vi "BSD Filename Header Formation.vi"(11 "Pre File F_Name":string) -> (3 "Head for BNAL":string)   [LabVIEW 2018]
panel:
  out "String":string
  out "Array":string[](array[string])
  out "after substring":string
  out "部分文字列の後":string
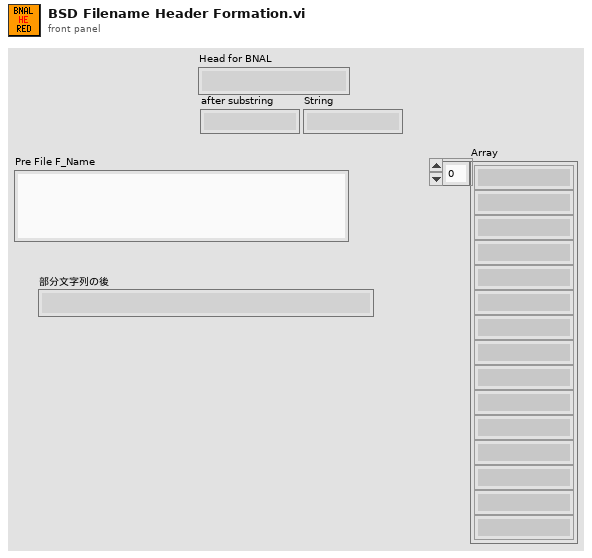
[diagram p1: front panel]
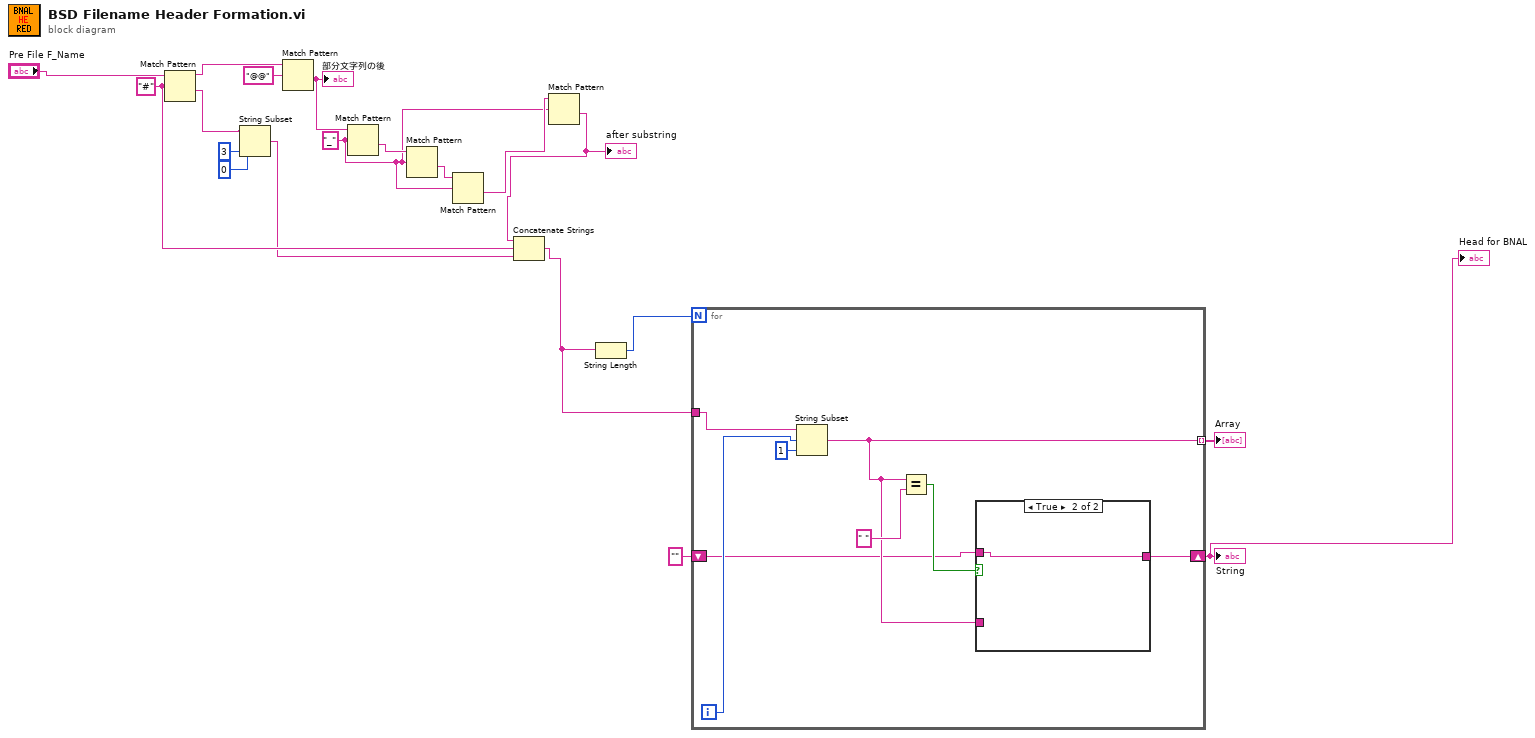
[diagram p0: block diagram]
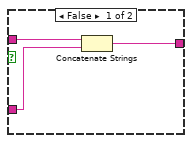
[diagram p2: hidden frame]
diagram:
  w7 = "_" ("正規表現")
  w10 = "#" ("正規表現")
  n1 = Match Pattern(string="Pre File F_Name", regular expression=w10) -> (before substring=w18:string, after substring=w13:string)  [unwired: 1 in, 2 out]
  n2 = String Subset(string=w13, offset (0)=0 ("オフセット（0）"), length (rest)=3 ("長さ（残り）")) -> (substring=w9:string)
  n3 = Match Pattern(string=w18, regular expression="@@" ("正規表現")) -> (after substring=w16:string)  [unwired: 1 in, 3 out]
  "部分文字列の後" <- w16
  n4 = Match Pattern(string=w16, regular expression=w7) -> (after substring=w15:string)  [unwired: 1 in, 3 out]
  n5 = Match Pattern(string=w15, regular expression=w7) -> (after substring=w14:string)  [unwired: 1 in, 3 out]
  n6 = Match Pattern(string=w14, regular expression=w7) -> (after substring=w8:string)  [unwired: 1 in, 3 out]
  n7 = Match Pattern(string=w8, regular expression=w7) -> (after substring=w6:string)  [unwired: 1 in, 3 out]
  "after substring" <- w6
  n8 = Concatenate Strings(w6, w10, w9) -> (w4:string)
  n9 = String Length(string=w4) -> (length=w5:i32)
  n10 = for {
    N: w5 -> [_]
    tunnel: w4 -> [w25]
    tunnel: [w22] -> w3 mode=indexing
    shift-right: [w21] -> w1
    shift-left: "" -> [w20]
    i -> [w26]
    n11 = String Subset(string=w25, offset (0)=w26, length (rest)=1 ("length (rest)")) -> (substring=w22:string)
    n12 = Equal?(x=w22, y=" ") -> (x = y?=w23:bool)
    n13 = case shown="True" w23 {
      tunnel: w22 -> [w30 _]
      tunnel: [w29 w31] -> w21
      tunnel: w20 -> [w28 w31]
      frame False {
        n14 = Concatenate Strings(w28, w30) -> (w29:string)
      }
      frame True {
      }
    }
  }
  "Head for BNAL" <- w1
  "Array" <- w3
  "String" <- w1
